vi "Zad2.vi"() -> ()   [LabVIEW 2025]
panel:
  in  "Password":string
  out "Valid":bool
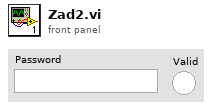
[diagram p1: front panel]
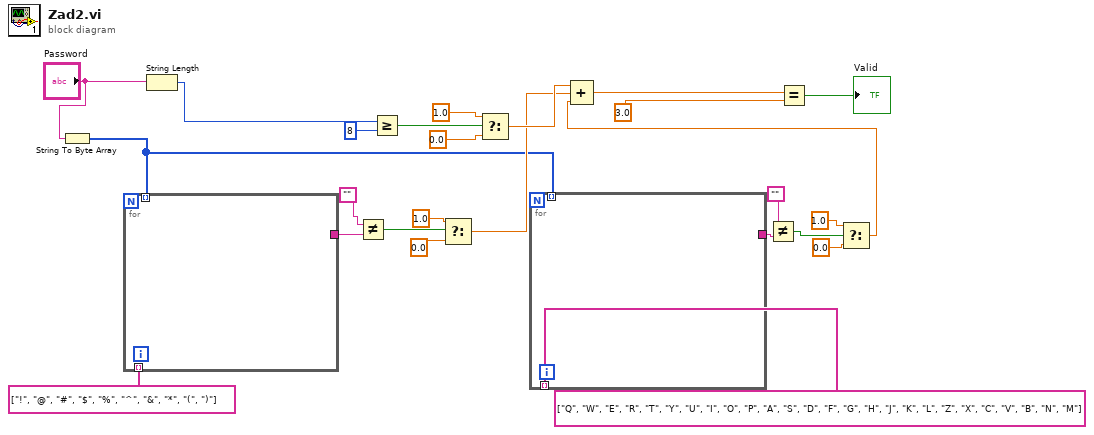
[diagram p0: block diagram]
diagram:
  n1 = String To Byte Array(string="Password") -> (unsigned byte array=w1:u8[])
  n2 = for {
    tunnel: w1 -> [_] mode=indexing
    tunnel: string[] ["!", "@", "#", "$", "%", "^", "&", "*", "(", ")"] ("regular expression") -> [_] mode=indexing
    tunnel: [_] -> w13
  }
  n3 = String Length(string="Password") -> (length=w25:i32)
  n4 = Not Equal?(x="", y=w13) -> (x != y?=w9:bool)
  n5 = Greater Or Equal?(x=w25, y=8) -> (x >= y?=w21:bool)
  n6 = Select(t=1.0, s=w9, f=0.0) -> (s? t:f=w4:dbl)
  n7 = Select(t=1.0, s=w21, f=0.0) -> (s? t:f=w18:dbl)
  n8 = for {
    tunnel: w1 -> [_] mode=indexing
    tunnel: string[] ["Q", "W", "E", "R", "T", "Y", "U", "I", "O", "P", "A", "S", "D", "F", "G", "H", "J", "K", "L", "Z", "X", "C", "V", "B", "N", "M"] ("regular expression") -> [_] mode=indexing
    tunnel: [_] -> w12
  }
  n9 = Not Equal?(x="", y=w12) -> (x != y?=w10:bool)
  n10 = Select(t=1.0, s=w10, f=0.0) -> (s? t:f=w3:dbl)
  n11 = Compound Arithmetic op=ADD(w18, w4, w3) -> (w17:dbl)
  n12 = Equal?(x=w17, y=3.0) -> (x = y?=→"Valid":bool)
